vi "demo.vi"() -> ()   [LabVIEW 2017]
uses:
  xono2l-build/Release/xono2l.dll
panel:
  out "error out":errorcluster
  in  "IP address of device":string="XXX.XXX.XXX.XXX"
  out "FRAMES UPDATING":bool
  out "ACQUIRING":bool
  out "CONNECTED":bool
  out "Acquisition frame rate":dbl
  out "US probe freq (MHz)":dbl format="%_3g"
  out "Depth (cm)":dbl
  out "DATA STATUS":u8
  out "US IMAGE":u8[][](graph)
  in  "?":bool
  out "Height":u32
  out "Width":u32
  in  "IP address":string="xxx.xxx.xxx.xxx"
  # "US Machine"
  # "US Frame"
  # "Frame capture DLL"
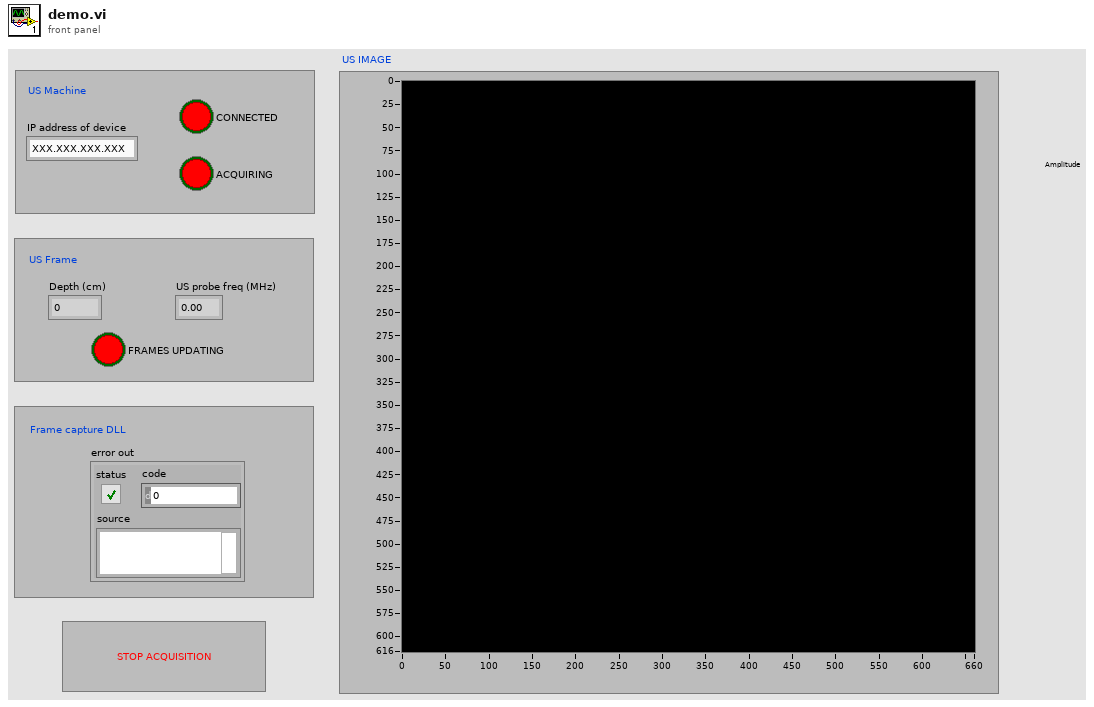
[diagram p1: front panel]
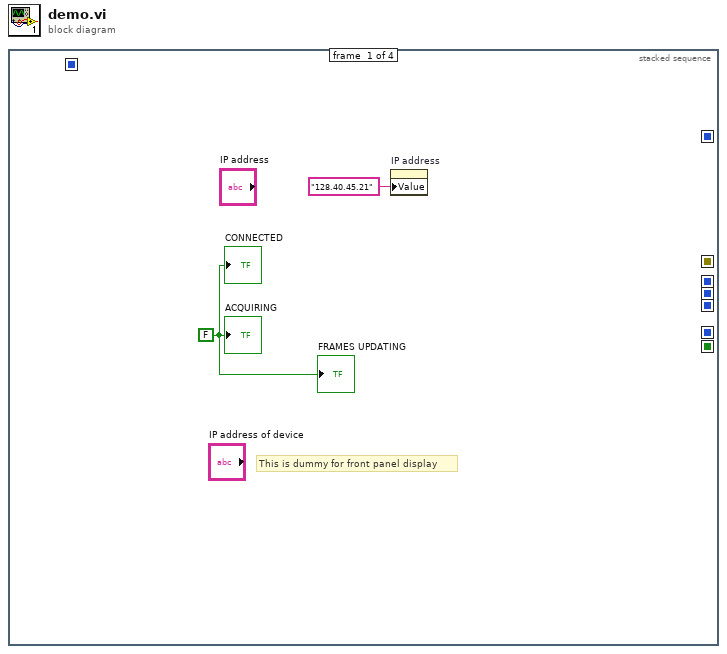
[diagram p0: block diagram]
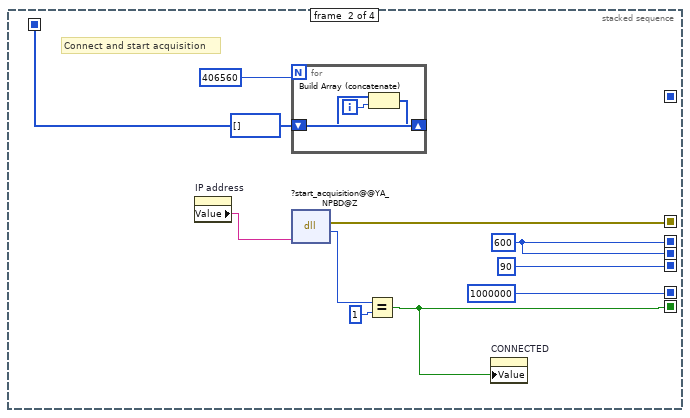
[diagram p2: hidden frame]
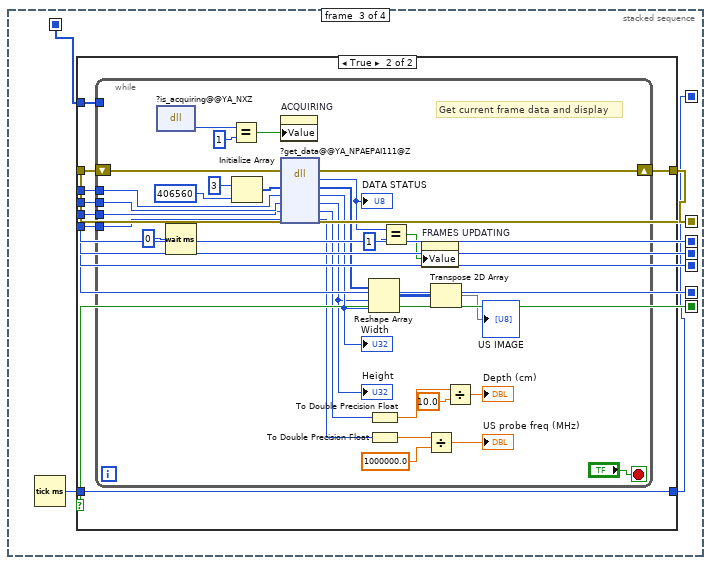
[diagram p3: hidden frame]
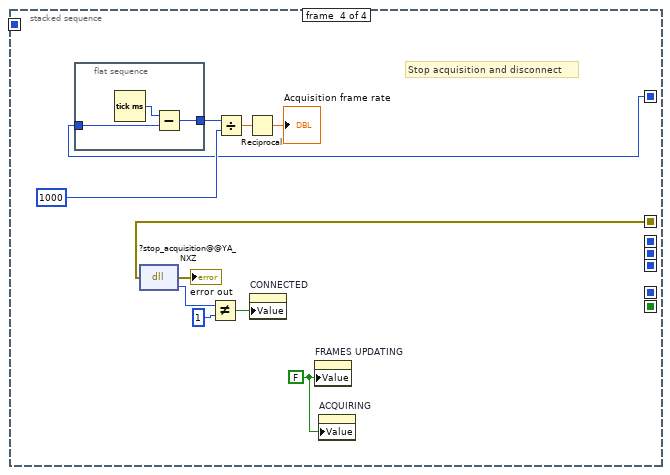
[diagram p5: hidden frame]
diagram:
  n1 = stacked-sequence {
    seq-local: [_ w13 _ _] -> [_ _ w25 _]
    seq-local: [_ w3 _ _] -> [_ _ w24 _]
    seq-local: [_ w5 _ _] -> [_ _ w23 _]
    seq-local: [_ w5 _ _] -> [_ _ w22 _]
    seq-local: [_ w9 _ _] -> [_ _ w21 _]
    seq-local: [_ u32 90 _ _] -> [_ _ w20 _]
    seq-local: [_ u32 1000000 _ _] -> [_ _ w19 _]
    seq-local: [_ _ w26 _] -> [_ _ _ w77]
    seq-local: [_ _ w17 _] -> [_ _ _ w72]
    frame #0 {
      w2 = FALSE
      # "This is dummy for front panel display"
      n2 = property on="IP address" class="Str"("Value"="128.40.45.21") -> ()  [unwired: 2 in, 2 out]
      "CONNECTED" <- w2
      "ACQUIRING" <- w2
      "FRAMES UPDATING" <- w2
    }
    frame #1 {
      w5 = u32 600 ("width")
      # "Connect and start acquisition"
      n3 = property on="IP address" class="Str"() -> ("Value"=w4:string)  [unwired: 2 in, 2 out]
      n4 = for {
        N: 406560 -> [_]
        shift-right: [w14] -> w9
        shift-left: i32[] [] -> [w16]
        i -> [w15]
        n5 = Build Array (concatenate)(w16, w15) -> (w14:i32[])
      }
      n6 = dll-call lib="J:/xono2l-build/Release/xono2l.dll" fn="?start_acquisition@@YA_NPBD@Z"("ip_address"=w4) -> (error out=w13:errorcluster, "return type"=w11:u8)  [unwired: 4 in, 1 out]
      n7 = Equal?(x=w11, y=u8 1) -> (x = y?=w3:bool)
      n8 = property on="CONNECTED" class="Bool (strict)"("Value"=w3) -> ()  [unwired: 2 in, 2 out]
    }
    frame #2 {
      n9 = Tick Count (ms)() -> (millisecond timer value=w18:u32)
      n10 = case shown="True" w24 {
        tunnel: w25 -> [w28 w36]
        tunnel: [w28 w35] -> w26
        tunnel: w23 -> [_ w34]
        tunnel: w22 -> [_ w33]
        tunnel: w21 -> [_ w32]
        tunnel: w20 -> [_ w31]
        tunnel: w19 -> [_ w30]
        tunnel: w18 -> [w27 w29]
        tunnel: [w27 w29] -> w17
        frame False {
        }
        frame True {
          n11 = while {
            tunnel: w34 -> [w64]
            tunnel: w33 -> [w63]
            tunnel: w32 -> [_]
            tunnel: w31 -> [w62]
            tunnel: w30 -> [w61]
            shift-right: [w65] -> w35
            shift-left: w36 -> [w66]
            stop <- "?" stop-if-true
            # "Get current frame data and display"
            n12 = dll-call lib="J:/xono2l-build/Release/xono2l.dll" fn="?is_acquiring@@YA_NXZ"() -> ("return type"=w42:u8)  [unwired: 3 in, 2 out]
            n13 = Wait (ms)(milliseconds to wait=u32 0) -> ()  [unwired: 1 out]
            n14 = Equal?(x=w42, y=u8 1) -> (x = y?=w40:bool)
            n15 = Initialize Array(u8 3 ("element"), 406560 ("dimension size")) -> (w55:u8[])
            n16 = property on="ACQUIRING" class="Bool (strict)"("Value"=w40) -> ()  [unwired: 2 in, 2 out]
            n17 = dll-call lib="J:/xono2l-build/Release/xono2l.dll" fn="?get_data@@YA_NPAEPAI111@Z"(error in=w66, "data"=w55, "width"=w64, "height"=w63, "depth"=w62, "freq"=w61) -> (error out=w65:errorcluster, "return type"=w39:u8, "data"=w53:u8[], "width"=w58:u32, "height"=w57:u32, "depth"=w44:u32, "freq"=w48:u32)  [unwired: 2 in, 1 out]
            "Width" <- w58
            "Height" <- w57
            "DATA STATUS" <- w39
            n18 = Reshape Array(w53, w57, w58) -> (w59:u8[][])
            n19 = To Double Precision Float(number=w44) -> (double precision float=w46:dbl)
            n20 = To Double Precision Float(number=w48) -> (double precision float=w47:dbl)
            n21 = Equal?(x=w39, y=u8 1) -> (x = y?=w37:bool)
            n22 = property on="FRAMES UPDATING" class="Bool (strict)"("Value"=w37) -> ()  [unwired: 2 in, 2 out]
            n23 = Divide(x=w47, y=1000000.0) -> (x/y=→"US probe freq (MHz)":dbl)
            n24 = Transpose 2D Array(2D array=w59) -> (transposed array=→"US IMAGE":u8[][])
            n25 = Divide(x=w46, y=10.0) -> (x/y=→"Depth (cm)":dbl)
          }
        }
      }
    }
    frame #3 {
      w68 = FALSE
      # "Stop acquisition and disconnect"
      n26 = flat-sequence {
        tunnel: [w79] -> w74
        tunnel: w72 -> [w78]
        frame #0 {
          n27 = Tick Count (ms)() -> (millisecond timer value=w80:u32)
          n28 = Subtract(x=w80, y=w78) -> (x-y=w79:u32)
        }
      }
      n29 = dll-call lib="J:/xono2l-build/Release/xono2l.dll" fn="?stop_acquisition@@YA_NXZ"(error in=w77) -> (error out=→"error out":errorcluster, "return type"=w71:u8)  [unwired: 2 in, 1 out]
      n30 = Not Equal?(x=w71, y=u8 1) -> (x != y?=w69:bool)
      n31 = Divide(x=w74, y=u32 1000) -> (x/y=w75:dbl)
      n32 = Reciprocal(x=w75) -> (1/x=→"Acquisition frame rate":dbl)
      n33 = property on="CONNECTED" class="Bool (strict)"("Value"=w69) -> ()  [unwired: 2 in, 2 out]
      n34 = property on="FRAMES UPDATING" class="Bool (strict)"("Value"=w68) -> ()  [unwired: 2 in, 2 out]
      n35 = property on="ACQUIRING" class="Bool (strict)"("Value"=w68) -> ()  [unwired: 2 in, 2 out]
    }
  }
